vi "Find InstrumentStudio Window.vi"(8 "error in":errorcluster, 11 "Top Window":u32) -> (0 "error out":errorcluster, 2 "IS Window Found?":bool, 3 "hWnd":u32)   [LabVIEW 2019, in "Screenshot Utility.lvlib"]
uses:
  Screenshot Utility.lvlib
  User32.dll
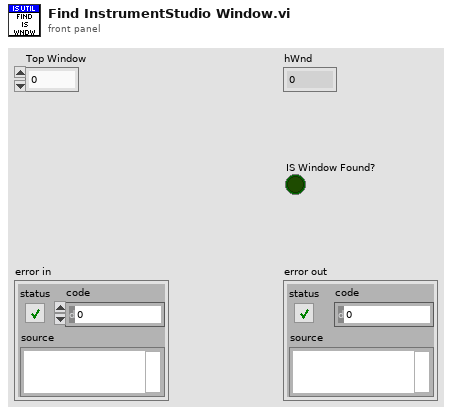
[diagram p1: front panel]
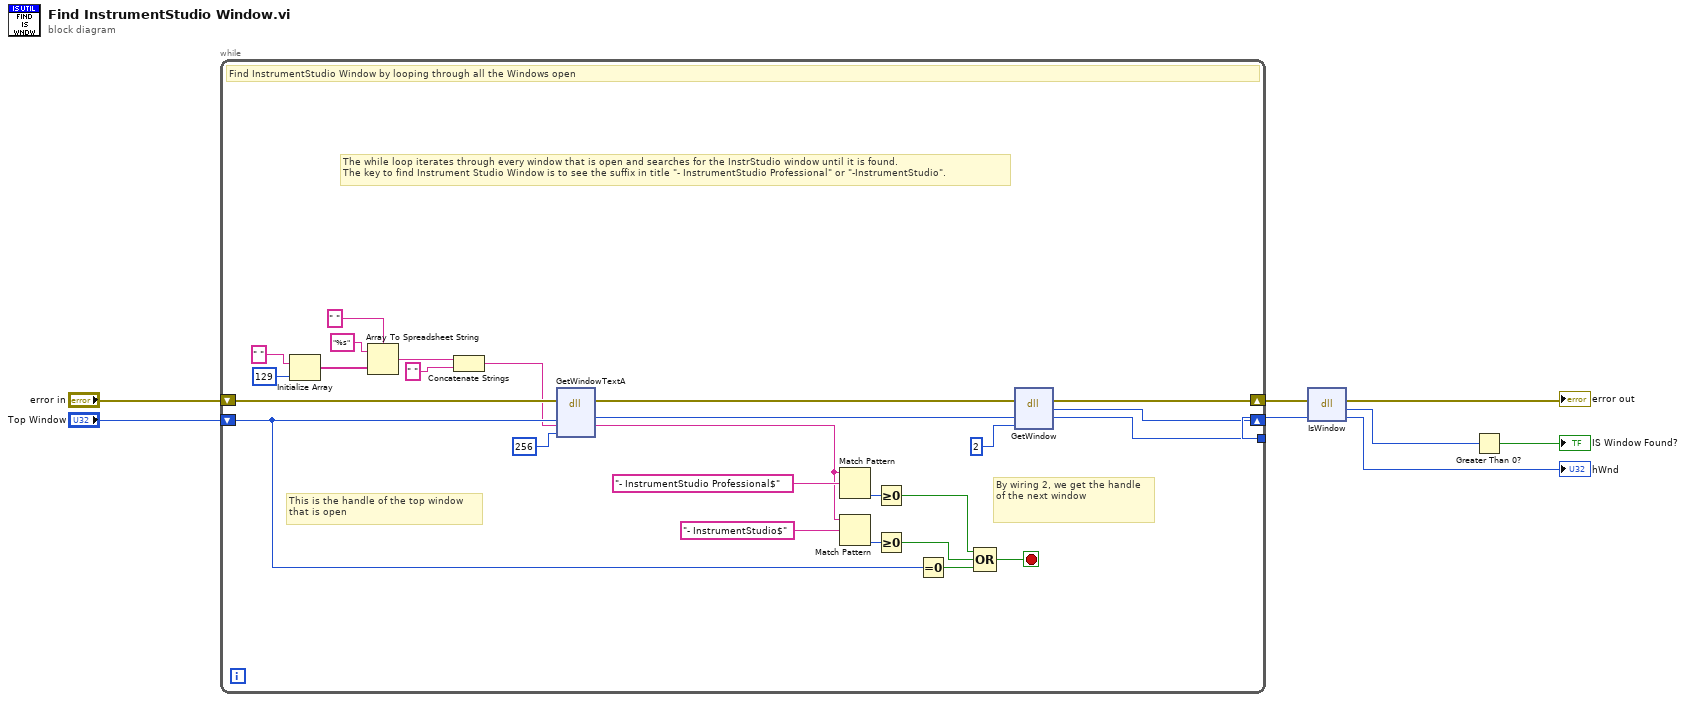
[diagram p0: block diagram]
diagram:
  n1 = while {
    shift-right: [w11] -> w6
    shift-left: "error in" -> [w33]
    shift-right: [w10] -> _
    shift-left: "Top Window" -> [w31]
    tunnel: [w9] -> w4
    stop <- w13 stop-if-true
    # "By wiring 2, we get the handle of the next window"
    # "This is the handle of the top window\nthat is open"
    # "The while loop iterates through every window that is open and searches for the InstrStudio window until it is found. \nThe key to find Instrument Studio Window is to see the suffix in title \"- InstrumentStudio Professional\" or \"-InstrumentStudio\"."
    # "Find InstrumentStudio Window by looping through all the Windows open"
    n2 = Initialize Array(" " ("lpExeName"), 129 ("dimension size")) -> (w28:string[])
    n3 = Array To Spreadsheet String(delimiter (Tab)=" ", array=w28, 3:"%s" ("format string")) -> (spreadsheet string=w24:string)
    n4 = Concatenate Strings(w24, " " ("string")) -> (w23:string)
    n5 = dll-call lib="USER32.DLL" fn="GetWindowTextA"(error in=w33, "hWnd"=w31, "IpString"=w23, "nMaxCount"=256) -> (error out=w19:errorcluster, "hWnd"=w20:u32, "IpString"=w12:string)  [unwired: 2 in, 3 out]
    n6 = Match Pattern(string=w12, regular expression="- InstrumentStudio Professional$") -> (offset past match=w21:i32)  [unwired: 1 in, 3 out]
    n7 = Match Pattern(string=w12, regular expression="- InstrumentStudio$") -> (offset past match=w17:i32)  [unwired: 1 in, 3 out]
    n8 = Greater Or Equal To 0?(x=w21) -> (x >= 0?=w16:bool)
    n9 = Greater Or Equal To 0?(x=w17) -> (x >= 0?=w15:bool)
    n10 = Equal To 0?(x=w31) -> (x = 0?=w14:bool)
    n11 = Compound Arithmetic op=OR(w16, w15, w14) -> (w13:bool)
    n12 = dll-call lib="USER32.DLL" fn="GetWindow"(error in=w19, "hWnd"=w20, "uCmd"=u32 2) -> (error out=w11:errorcluster, "return"=w10:u32, "hWnd"=w9:u32)  [unwired: 2 in, 2 out]
  }
  n13 = dll-call lib="USER32.DLL" fn="IsWindow"(error in=w6, "hWnd"=w4) -> (error out=→"error out":errorcluster, "return"=w2:u32, "hWnd"=→"hWnd":u32)  [unwired: 2 in, 1 out]
  n14 = Greater Than 0?(x=w2) -> (x > 0?=→"IS Window Found?":bool)
